vi "AS_Load_receip.vi"(8 "error in":errorcluster) -> (0 "error out":errorcluster, 3 "S array":T2(array[cluster]))   [LabVIEW 2018]
panel:
  out "stripped path":path
  in  "index":i32
  out "ACond#":i32
  out "S New Info and MiN out":T1={"Sample Sequence"="GATGATGATGATGATGAT", "Right Read MIN"=6, "Filter P"=0, "STD Type"=enum."Region", "Base Table"=[], "Selection"=enum."10kHz", "noise MAX"=3, "Sample name"=""} {"Base Table"."Value 3" format="%.2g"}
  out "appended path":path
  in  "Receip Name":u16(ring) items=["2018_1002_055233.tdms", "2018_1002_055233_TO.tdms", "2018_1004_134258_TO64.tdms", "2018_1029_121133_mAset.tdms", "2018_1029_150003_mAtruset.tdms", "2018_1113_100053_Msan.tdms", "2019_0722_135800_ini.tdms", "2020_0428_105016_To22.tdms", "2020_0722_144051_20200722_TO.tdms", "2020_0728_130619_TO.tdms", "2020_0728_181704_tto.tdms", "2020_0729_180356_tyy.tdms", "2020_0729_183711_TT.tdms", "2020_0729_184713_TTT.tdms", "2020_0811_144904_RRRR.tdms", "2020_0819_014005_TOR.tdms", "2020_1224_122246_tttt.tdms", "2021_0420_154433_MYC (OOO TTT の競合コピー 2021-04-21).tdms", "2021_0420_154433_MYC.tdms", "2022_1029_183743_CpG.tdms", "2022_1102_113057_new.tdms"]
  in  "Set":bool
  out "Array 2":string[](array[string])
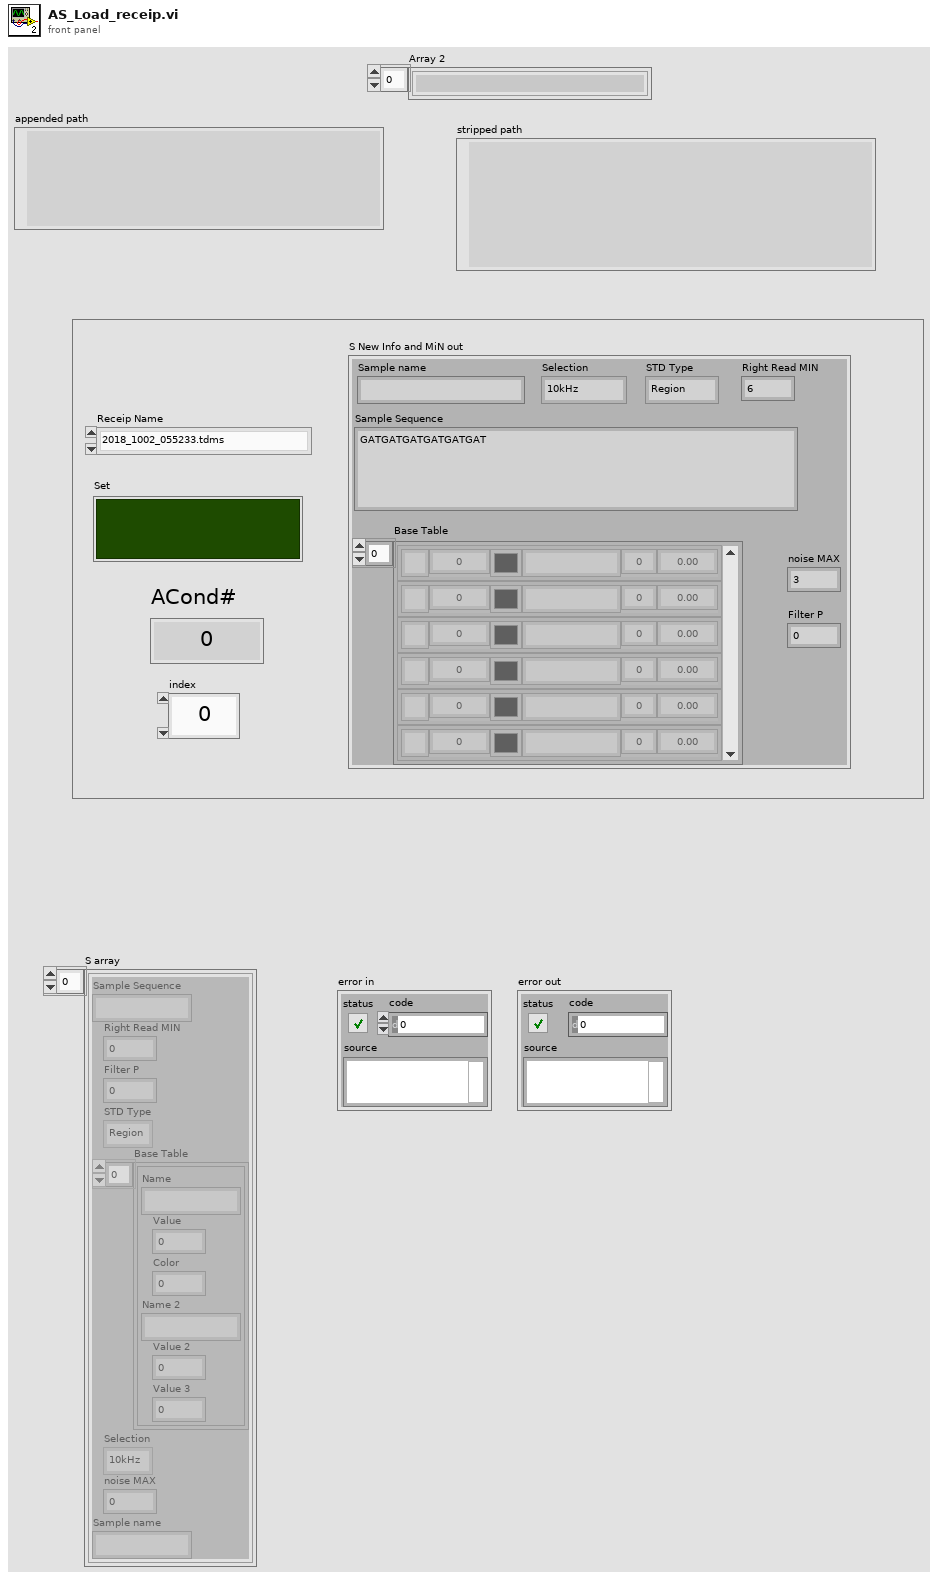
[diagram p1: front panel]
types:
  T1 = cluster{"Sample Sequence":string, "Right Read MIN":i32, "Filter P":i32, "STD Type":enum16{"Region", "Each", "Fixed"}, "Base Table":cluster{"Name":string, "Value":dbl, "Color":u32, "Name 2":string, "Value 2":dbl, "Value 3":dbl}[], "Selection":enum16{"10kHz", "100kHz"}, "noise MAX":i32, "Sample name":string}
  T2 = cluster{"Sample Sequence":string, "Right Read MIN":i32, "Filter P":i32, "STD Type":enum16{"Region", "Each", "Fixed"}, "Base Table":cluster{"Name":string, "Value":dbl, "Color":u32, "Name 2":string, "Value 2":dbl, "Value 3":dbl}[], "Selection":enum16{"10kHz", "100kHz"}, "noise MAX":i32, "Sample name":string}[]
  T3 = cluster{"Sample Sequence":string, "Right Read MIN":i32, "Filter P":i32, "STD Type":enum16{"Region", "Each", "Fixed"}, "Base Table":cluster{"Base":string, "RC_value":dbl, "Color":u32, "Base_N":string, "Base#":dbl, "STD":dbl}[], "Selection":enum16{"10kHz", "100kHz"}, "noise MAX":i32, "Sample name":string}[]
  T4 = cluster{"Sample Sequence":string, "Right Read MIN":i32, "Filter P":i32, "STD Type":enum16{"Region", "Each", "Fixed"}, "Base Table":cluster{"Base":string, "RC_value":dbl, "Color":u32, "Base_N":string, "Base#":dbl, "STD":dbl}[], "Selection":enum16{"10kHz", "100kHz"}, "noise MAX":i32, "Sample name":string}
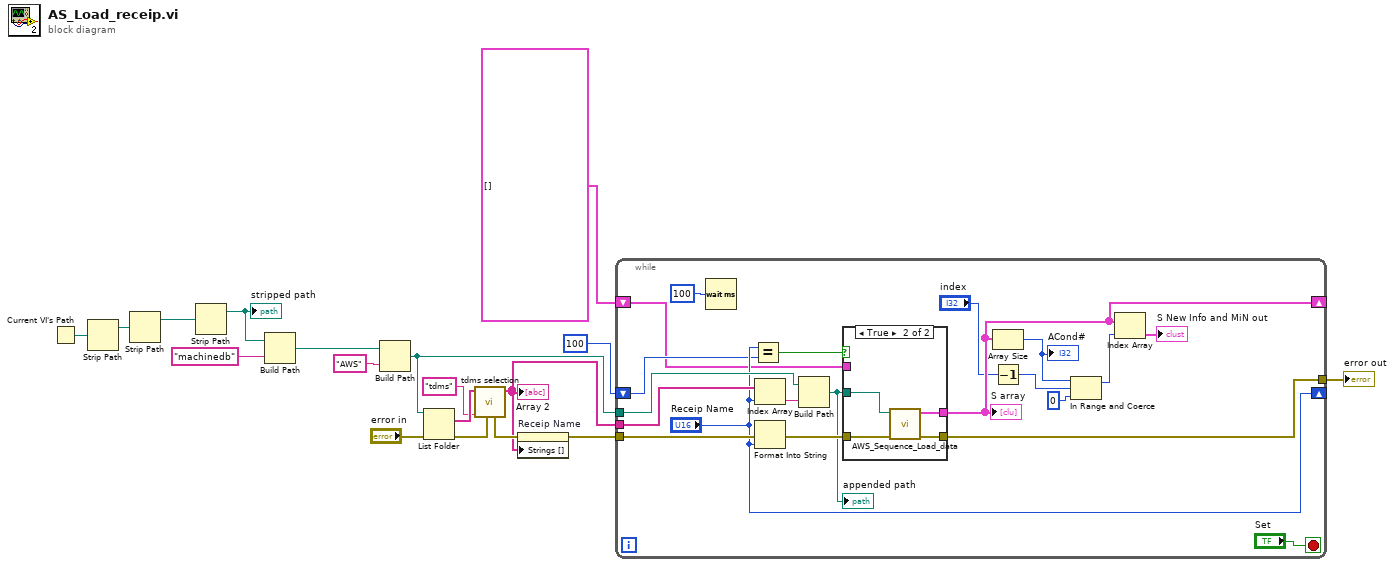
[diagram p0: block diagram]
diagram:
  n1 = Current VI's Path() -> (path=w8:path)
  n2 = Strip Path(path=w8) -> (stripped path=w7:path)  [unwired: 1 out]
  n3 = Strip Path(path=w7) -> (stripped path=w6:path)  [unwired: 1 out]
  n4 = Strip Path(path=w6) -> (stripped path=w5:path)  [unwired: 1 out]
  "stripped path" <- w5
  n5 = Build Path(base path=w5, name or relative path="machinedb") -> (appended path=w3:path)
  n6 = Build Path(base path=w3, name or relative path="AWS") -> (appended path=w1:path)
  n7 = List Folder(path=w1, error in="error in") -> (filenames=w18:string[], error out=w16:errorcluster)  [unwired: 2 in, 2 out]
  n8 = call "tdms selection.vi"("error in"=w16, "string"="tdms", "Filename List"=w18) -> ("Array 2"=w11:string[], "error out"=w13:errorcluster)  [unwired: 6 in, 1 out]
  "Array 2" <- w11
  n9 = property on="Receip Name" class="Ring (strict)"(error in=w13, "Strings []"=w11) -> (error out=w12:errorcluster)  [unwired: 1 in, 1 out]
  n10 = while {
    tunnel: w12 -> [w37]
    tunnel: [w28] -> w14
    tunnel: w1 -> [w36]
    tunnel: w11 -> [w34]
    shift-right: ["Receip Name"] -> _
    shift-left: u16 100 ("Receip Name") -> [w31]
    shift-right: [w25] -> _
    shift-left: T2 [] -> [w26]
    stop <- "Set" stop-if-true
    n11 = Wait (ms)(milliseconds to wait=u32 100) -> ()  [unwired: 1 out]
    n12 = Equal?(x="Receip Name", y=w31) -> (x = y?=w30:bool)
    n13 = Index Array(array=w34, index="Receip Name") -> (element=w33:string)
    n14 = Format Into String(error in=w37, "Receip Name") -> (error out=w29:errorcluster)  [unwired: 2 in, 1 out]
    n15 = Build Path(base path=w36, name or relative path=w33) -> (appended path=w27:path)
    "appended path" <- w27
    n16 = case shown="True" w30 {
      tunnel: w29 -> [w40 w44]
      tunnel: [w40 w43] -> w28
      tunnel: w27 -> [_ w42]
      tunnel: [w39 w41] -> w25
      tunnel: w26 -> [w39 _]
      frame False {
      }
      frame True {
        n17 = call "AWS_Sequence_Load_data.vi"("error in"=w44, "appended path"=w42) -> ("error out"=w43:errorcluster, "S array"=w41:T3)  [unwired: 8 in]
      }
    }
    "S array" <- w25
    n18 = Array Size(array=w25) -> (size(s)=w19:i32)
    "ACond#" <- w19
    n19 = Decrement(x="index") -> (x-1=w21:i32)
    n20 = In Range and Coerce(upper limit=w19, x=w21, lower limit=0) -> (coerced(x)=w22:i32)  [unwired: 1 out]
    n21 = Index Array(array=w25, index=w22) -> (element=→"S New Info and MiN out":T4)
  }
  "error out" <- w14
